vi "Call Function.vi"(6 "Input String":string, 8 "error in":errorcluster, 9 "Function":string, 10 "Python Script":path, 11 "IPython Caller in":refnum<class "Mock IPython Caller.lvclass">) -> (0 "error out":errorcluster, 2 "Return String":string, 3 "IPython Caller out":refnum<class "Mock IPython Caller.lvclass">)   [LabVIEW 2026, in "Mock IPython Caller.lvclass"]
doc: "This VI calls the specified function from a python script. This VI can only call functions with a string input and output parameter. The function uses the tool global virtual environment."
uses:
  Mock IPython Caller.lvclass
  C:/Program Files/National Instruments/LabVIEW 2026/vi.lib/Astemes/LMock/Mock.lvclass
  Mock IPython Caller.lvclass/Mock IPython Caller.ctl
  <vilib>/Astemes/LMock/Mock.lvclass
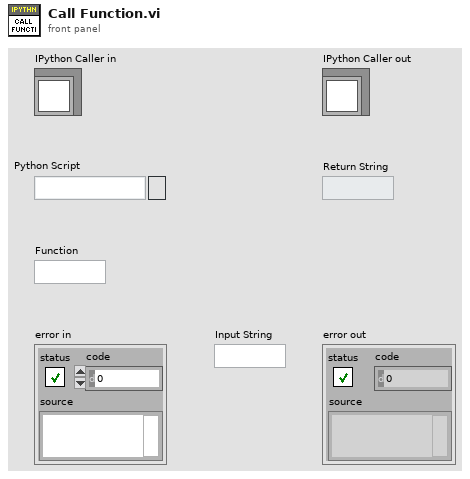
[diagram p1: front panel]
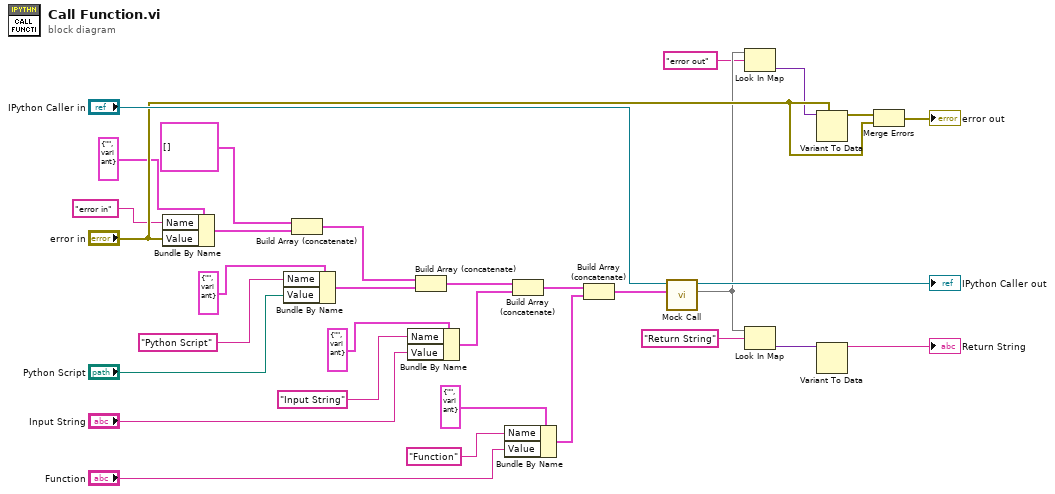
[diagram p0: block diagram]
diagram:
  n1 = Bundle By Name(cluster=cluster{"Name":string, "Value":variant} {"Name"="", "Value"=variant} ("element"), "Name"="error in", "Value"="error in") -> (w7:cluster{"Name":string, "Value":variant})
  n2 = Bundle By Name(cluster=cluster{"Name":string, "Value":variant} {"Name"="", "Value"=variant} ("element"), "Name"="Python Script", "Value"="Python Script") -> (w5:cluster{"Name":string, "Value":variant})
  n3 = Build Array (concatenate)(cluster{"Name":string, "Value":variant}[] [] ("Control Values"), w7) -> (w19:cluster{"Name":string, "Value":variant}[])
  n4 = Bundle By Name(cluster=cluster{"Name":string, "Value":variant} {"Name"="", "Value"=variant} ("element"), "Name"="Input String", "Value"="Input String") -> (w3:cluster{"Name":string, "Value":variant})
  n5 = Build Array (concatenate)(w19, w5) -> (w22:cluster{"Name":string, "Value":variant}[])
  n6 = Bundle By Name(cluster=cluster{"Name":string, "Value":variant} {"Name"="", "Value"=variant} ("element"), "Name"="Function", "Value"="Function") -> (w1:cluster{"Name":string, "Value":variant})
  n7 = Build Array (concatenate)(w22, w3) -> (w25:cluster{"Name":string, "Value":variant}[])
  n8 = Build Array (concatenate)(w25, w1) -> (w28:cluster{"Name":string, "Value":variant}[])
  n9 = call <vilib>:"Mock Call.vi"("Control Values"=w28, "Mock In"="IPython Caller in") -> ("Return Values"=w17:map{string, variant}, "Mock Out"=→"IPython Caller out":refnum<class "Mock IPython Caller.lvclass">)  [unwired: 8 in]
  n10 = Look In Map(map=w17, key="error out") -> (value=w12:variant)  [unwired: 1 in, 1 out]
  n11 = Look In Map(map=w17, key="Return String") -> (value=w15:variant)  [unwired: 1 in, 1 out]
  n12 = Variant To Data(type="error in", Variant=w12) -> (data=w11:errorcluster)  [unwired: 1 in, 1 out]
  n13 = Variant To Data(Variant=w15) -> (data=→"Return String":string)  [unwired: 2 in, 1 out]
  n14 = Merge Errors(w11, "error in") -> (→"error out":errorcluster)
